vi "initialize.vi"(8 "error in":errorcluster, 10 "Target Configuration":refnum<class "PL_Target Configuration.lvclass">, 11 "Target Runtime in":refnum<class "PL_Target Runtime.lvclass">) -> (0 "error out":errorcluster, 3 "Target Runtime out":refnum<class "PL_Target Runtime.lvclass">)   [LabVIEW 2013, in "PL_Target Runtime.lvclass"]
doc: "Initializes a target runtime object with a target configuration. This includes initializing target-wide behavior (like loading a bitfile) and caching any associated information or references. Only one target should be initialized per LabVIEW context, and generally only one should be used per hardware device."
uses:
  PL_Target Runtime.lvclass
  target configuration/PL_Target Configuration.lvclass
  target configuration/PL_Target Configuration.lvclass/PL_Target Configuration.ctl
  PL_Target Runtime.lvclass/PL_Target Runtime.ctl
  target configuration/Read load bitfile.vi
  target configuration/Read RIO FPGA.vi
  target configuration/Read bitfile path.vi
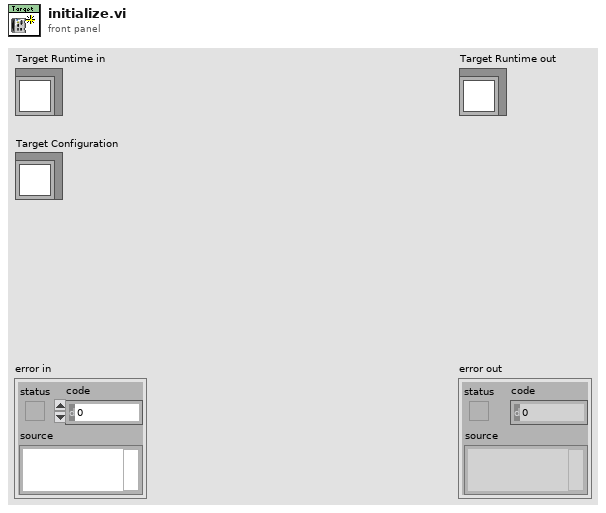
[diagram p1: front panel]
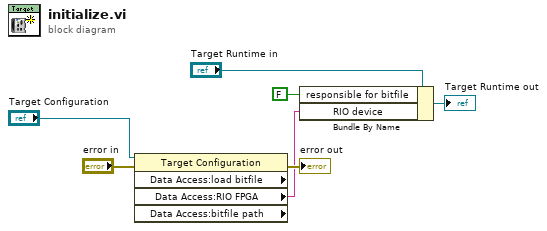
[diagram p0: block diagram]
diagram:
  n1 = property class="Target Configuration" props=["Data Access:load bitfile", "Data Access:RIO FPGA", "Data Access:bitfile path"](reference="Target Configuration", error in="error in") -> (error out=→"error out":errorcluster, "Data Access:RIO FPGA"=w2:string)  [unwired: 3 out]
  n2 = Bundle By Name(cluster="Target Runtime in", "responsible for bitfile"=FALSE, "RIO device"=w2) -> (→"Target Runtime out":refnum<class "PL_Target Runtime.lvclass">)
